vi "Echo_Handle_Frames.vi"(5 "buffers":T2, 6 "result":T1, 7 "context":T3 {"ack hi" format="%.0x"; "ack lo" format="%.0x"; "test hi" format="%.0x"; "test lo" format="%.0x"}, 8 "error in (no error)":errorcluster, 9 "counters in":T4, 10 "time store in":T5, 11 "tx in":u8[](array[numeric])) -> (0 "error out":errorcluster, 1 "counters out":T4, 2 "time store out":T5, 3 "tx out":u8[](array[numeric]))   [LabVIEW 2021]
doc: "S5 echo: handles the frames of one W13 read. Test frame (ID in test range, not TX ack, = 3 bytes) ? echo with W14 at ID + echo offset, stores t_dev and the LabVIEW times at key = idx·65536 + seq. TX ack in the ack range ? 36-byte Echo_Report (big-endian) by UDP to the harness, entry cleared. Updates all counters. tx and time store are changed in place."
uses:
  Echo_Time_Store.ctl
  Echo_Counters.ctl
  Echo_Context.ctl
  C_RX_Buffers.ctl
  CANsub_C.lvlib
  C_Decode_Result.ctl
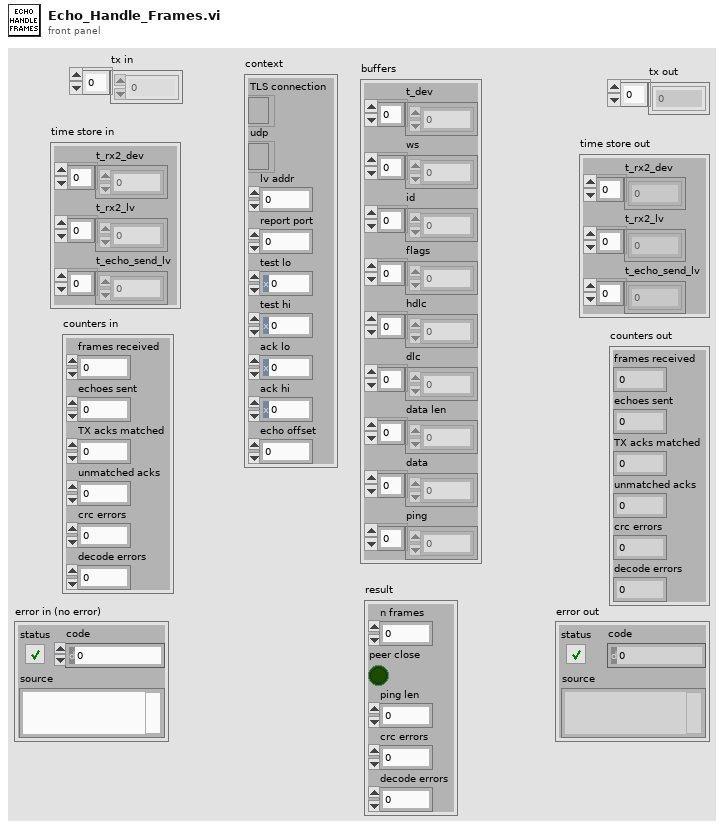
[diagram p1: front panel]
types:
  T1 = typedef "CANsub_C.lvlib/C_Decode_Result.ctl" = cluster{"n frames":i32, "peer close":bool, "ping len":i32, "crc errors":u32, "decode errors":i32}
  T2 = typedef "CANsub_C.lvlib/C_RX_Buffers.ctl" = cluster{"t_dev":dbl[], "ws":u8[], "id":u32[], "flags":u16[], "hdlc":u8[], "dlc":u8[], "data len":u8[], "data":u8[], "ping":u8[]}
  T3 = typedef "Echo_Context.ctl" = cluster{"TLS connection":refnum<k5>, "udp":refnum<k16>, "lv addr":u32, "report port":u16, "test lo":u32, "test hi":u32, "ack lo":u32, "ack hi":u32, "echo offset":i32}
  T4 = typedef "Echo_Counters.ctl" = cluster{"frames received":u32, "echoes sent":u32, "TX acks matched":u32, "unmatched acks":u32, "crc errors":u32, "decode errors":i32}
  T5 = typedef "Echo_Time_Store.ctl" = cluster{"t_rx2_dev":dbl[], "t_rx2_lv":dbl[], "t_echo_send_lv":dbl[]}
  T6 = typedef "Echo_Frame.ctl" = cluster{"kind":T7, "id":u32, "t_dev":dbl, "seq":u16, "idx":u8, "key":i32, "index":i32}
  T7 = typedef "Echo_Frame_Kind.ctl" = enum16{"Other", "Test", "Ack"}
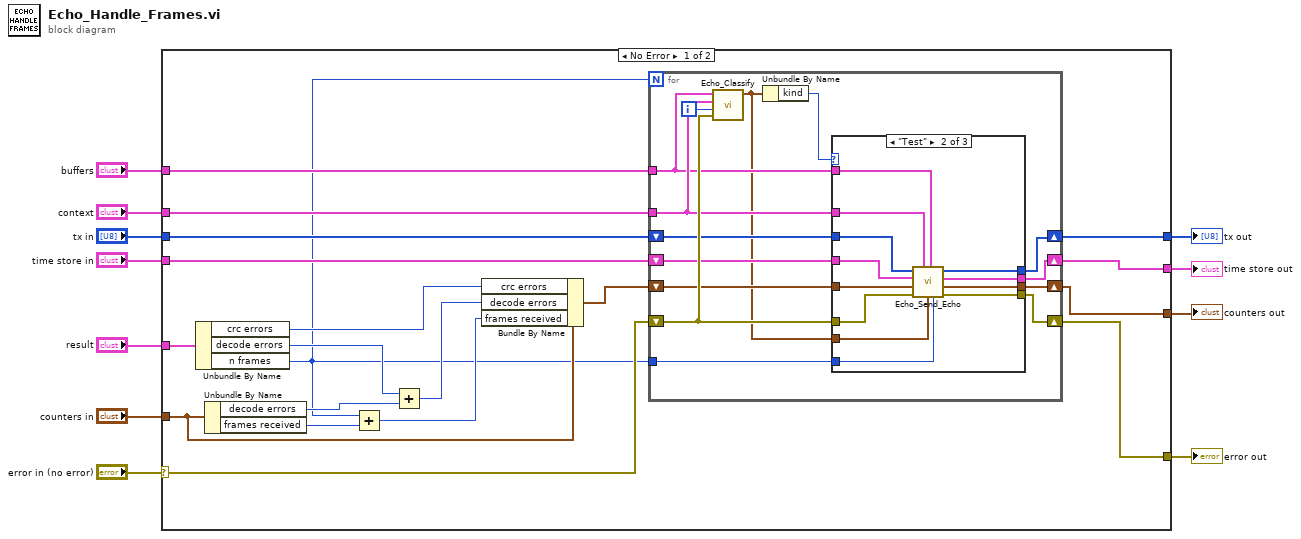
[diagram p0: block diagram]
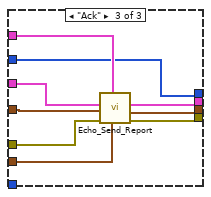
[diagram p3: hidden frame]
diagram:
  n1 = case shown="No Error" "error in (no error)" {
    selector: "error in (no error)" -> [w19 w73]
    tunnel: [w12 w73] -> w10
    tunnel: [w15 w72] -> w9
    tunnel: "tx in" -> [w22 w72]
    tunnel: [w14 w71] -> w7
    tunnel: "time store in" -> [w21 w71]
    tunnel: [w13 w70] -> w5
    tunnel: "counters in" -> [w29 w70]
    tunnel: "context" -> [w17 _]
    tunnel: "buffers" -> [w18 _]
    tunnel: "result" -> [w30 _]
    frame No Error {
      n2 = Unbundle By Name(w30) -> ("crc errors"=w27:u32, "decode errors"=w26:i32, "n frames"=w16:i32)
      n3 = Unbundle By Name(w29) -> ("decode errors"=w24:i32, "frames received"=w28:u32)
      n4 = Add(x=w16, y=w28) -> (x+y=w23:u32)
      n5 = Add(x=w26, y=w24) -> (x+y=w25:i32)
      n6 = Bundle By Name(cluster=w29, "crc errors"=w27, "decode errors"=w25, "frames received"=w23) -> (w20:T4)
      n7 = for {
        N: w16 -> [_]
        shift-right: [w34] -> w15
        shift-left: w22 -> [w39]
        shift-right: [w33] -> w14
        shift-left: w21 -> [w38]
        shift-right: [w31] -> w13
        shift-left: w20 -> [w37]
        shift-right: [w32] -> w12
        shift-left: w19 -> [w42]
        tunnel: w18 -> [w40]
        tunnel: w17 -> [w41]
        tunnel: w16 -> [w35]
        i -> [w44]
        n8 = call "Echo_Classify.vi"("error in (no error)"=w42, "i"=w44, "context"=w41, "buffers"=w40) -> ("frame"=w36:T6)  [unwired: 6 in, 1 out]
        n9 = Unbundle By Name(w36) -> ("kind"=w43:T7)
        n10 = case shown="\"Test\"" w43 {
          tunnel: [w48 w60 w61] -> w34
          tunnel: [w47 w59 w69] -> w33
          tunnel: [w46 w58 w68] -> w31
          tunnel: [w45 w57 w67] -> w32
          tunnel: w42 -> [w45 w56 w66]
          tunnel: w41 -> [_ w55 w64]
          tunnel: w40 -> [_ w54 _]
          tunnel: w39 -> [w48 w53 w61]
          tunnel: w38 -> [w47 w52 w63]
          tunnel: w37 -> [w46 w51 w65]
          tunnel: w36 -> [_ w50 w62]
          tunnel: w35 -> [_ w49 _]
          frame "Other", Default {
          }
          frame "Test" {
            n11 = call "Echo_Send_Echo.vi"("n frames"=w49, "buffers"=w54, "frame"=w50, "context"=w55, "error in (no error)"=w56, "counters in"=w51, "time store in"=w52, "tx in"=w53) -> ("error out"=w57:errorcluster, "counters out"=w58:T4, "time store out"=w59:T5, "tx out"=w60:u8[])
          }
          frame "Ack" {
            n12 = call "Echo_Send_Report.vi"("frame"=w62, "context"=w64, "error in (no error)"=w66, "counters in"=w65, "time store in"=w63) -> ("error out"=w67:errorcluster, "counters out"=w68:T4, "time store out"=w69:T5)  [unwired: 4 in]
          }
        }
      }
    }
    frame Error {
    }
  }
  "error out" <- w10
  "tx out" <- w9
  "time store out" <- w7
  "counters out" <- w5
